vi "upload_ingest.csv.vi"(4 "Properties":map{string, string}(c390), 6 "Labels":string[](array[string]), 7 "Timestamp SeriesName":string, 8 "error in":errorcluster, 10 "File Path":path, 11 "Nominal Client in":refnum<class "Nominal Client.lvclass">) -> (0 "error out":errorcluster, 2 "datasetRID":string, 3 "Nominal Client out":refnum<class "Nominal Client.lvclass">)   [LabVIEW 2020, in "Nominal Client.lvclass"]
doc: "Uploads a file to S3\nIngests video with common settings:\n - No TimeManifest (uses Start Timestamp and a scale factor of 1.\nNew Target: Name based on path name and timestamp"
uses:
  Nominal Client.lvclass
  datasources/dataset/dataset.lvclass
  nominal types/channelConfig/channelConfig.lvclass
  datasources/s3/s3.lvclass
  C:/code/labview-client/lv_src/datasources/source/source.lvclass
  datasources/source/create_s3.vi
  ts.iso8601/build.iso8601.vi
  datasources/target/create_new.vi
  ingest_csv.vi
  Nominal Client.lvclass/Nominal Client.ctl
  datasources/target/target.lvclass
  datasources/source/source.lvclass
  timestampMetadata/timestampMetadata.lvclass
  ts.iso8601/ts.iso8601.lvclass
  C:/code/labview-client/lv_src/datasources/payload/payload.lvclass
  C:/code/labview-client/lv_src/datasources/s3/s3.lvclass
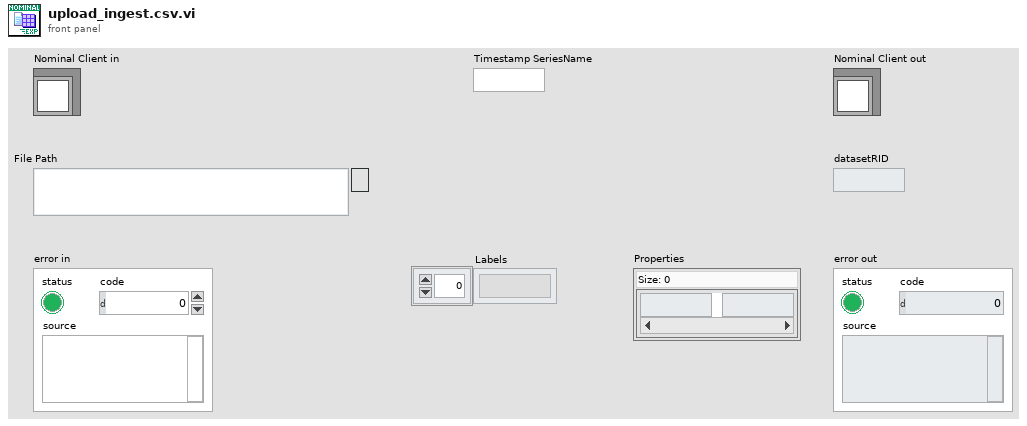
[diagram p1: front panel]
types:
  T1 = cluster{"dataset":refnum<class "dataset.lvclass">, "channelConfig":refnum<class "channelConfig.lvclass">}
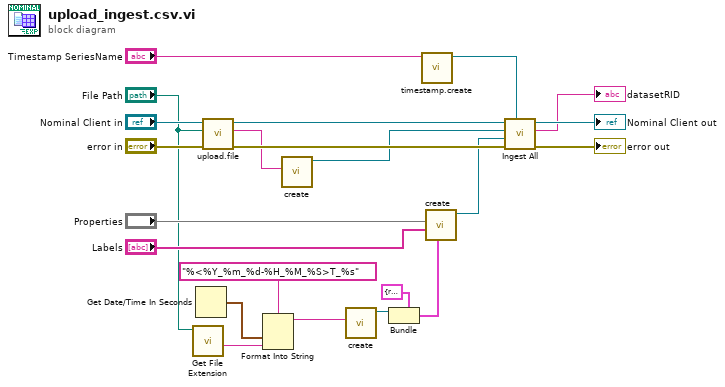
[diagram p0: block diagram]
diagram:
  n1 = call <vilib>:"Get File Extension.vi"("file"="File Path") -> ("filename without extension"=w6:string)  [unwired: 6 in, 4 out]
  n2 = Get Date/Time In Seconds() -> (seconds since 1Jan1904=w1:timestamp)
  n3 = call "upload.file.vi"("error in"="error in", "File"="File Path", "Nominal Client in"="Nominal Client in") -> ("error out"=w21:errorcluster, "Path to S3 File"=w19:string, "Nominal Client out"=w22:refnum<class "Nominal Client.lvclass">)  [unwired: 6 in]
  n4 = Format Into String(format string="%<%Y_%m_%d-%H_%M_%S>T_%s", w1, w6) -> (resulting string=w5:string)  [unwired: 2 in, 1 out]
  n5 = call-poly "create.vi"("Path"=w19) -> ("source"=w18:refnum<class "s3.lvclass">)  [unwired: 10 in]
  n6 = call "create.vi"("Name"=w5) -> ("dataset"=w16:refnum<class "dataset.lvclass">)  [unwired: 10 in]
  n7 = Bundle(cluster=T1 {"dataset"=refnum, "channelConfig"=refnum} ("Optional"), "dataset"=w16) -> (w15:T1)  [unwired: 1 in]
  n8 = call-poly "timestamp.create.vi"("seriesName"="Timestamp SeriesName") -> ("Timestamp Metadata"=w3:refnum<class "timestampMetadata.lvclass">)  [unwired: 10 in]
  n9 = call-poly "create.vi"("Optional"=w15, "Labels"="Labels", "Properties"="Properties") -> ("New Target"=w20:refnum<class "target.lvclass">)  [unwired: 8 in]
  n10 = call-poly "Ingest All.vi"("timestampMetadata"=w3, "error in"=w21, "Target"=w20, "Source"=w18, "Nominal Client in"=w22) -> ("error out"=→"error out":errorcluster, "datasetRid"=→"datasetRID":string, "Nominal Client out"=→"Nominal Client out":refnum<class "Nominal Client.lvclass">)  [unwired: 3 in, 1 out]
